vi "GDSProject_CreateFolder.vi"(0 "Project Refnum In":refnum<vi>, 1 "Project Item To Create Folder Below(Use MyComputer if not wired)":refnum<vi>, 3 "FolderName":string, 5 "error in (no error)":errorcluster, 7 "FolderScope":T1(array[ring]), 8 "CreateThePhysicalFolderIfPossible(False)":bool, 9 "GuessFolderScope(False)":bool) -> (14 "Project Refnum Out":refnum<vi>, 15 "ItemOut":refnum<vi>, 16 "FolderCreated":bool, 19 "error out":errorcluster)   [LabVIEW 2020]
panel:
  # "E.g. Private/SubPrivate"
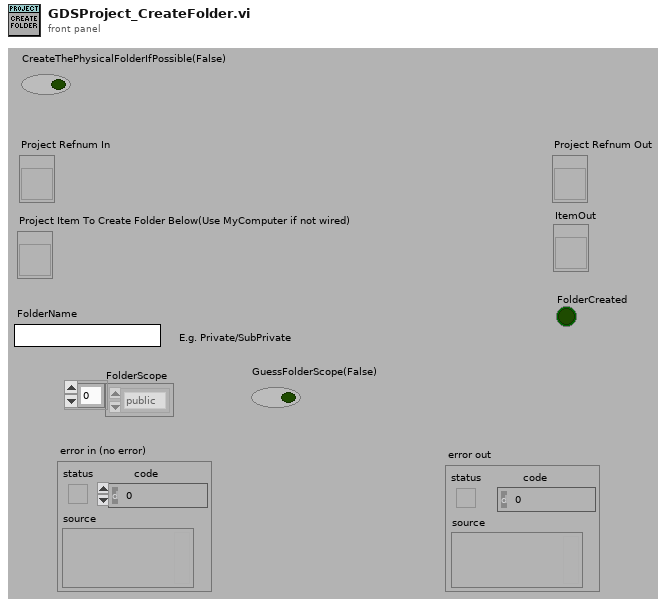
[diagram p1: front panel]
types:
  T1 = enum32{"invalid scope", "public", "private", "protected", "community"}[]
  T2 = enum32{"invalid scope", "public", "private", "protected"}
  T3 = enum32{"invalid scope", "public", "private", "protected", "community"}
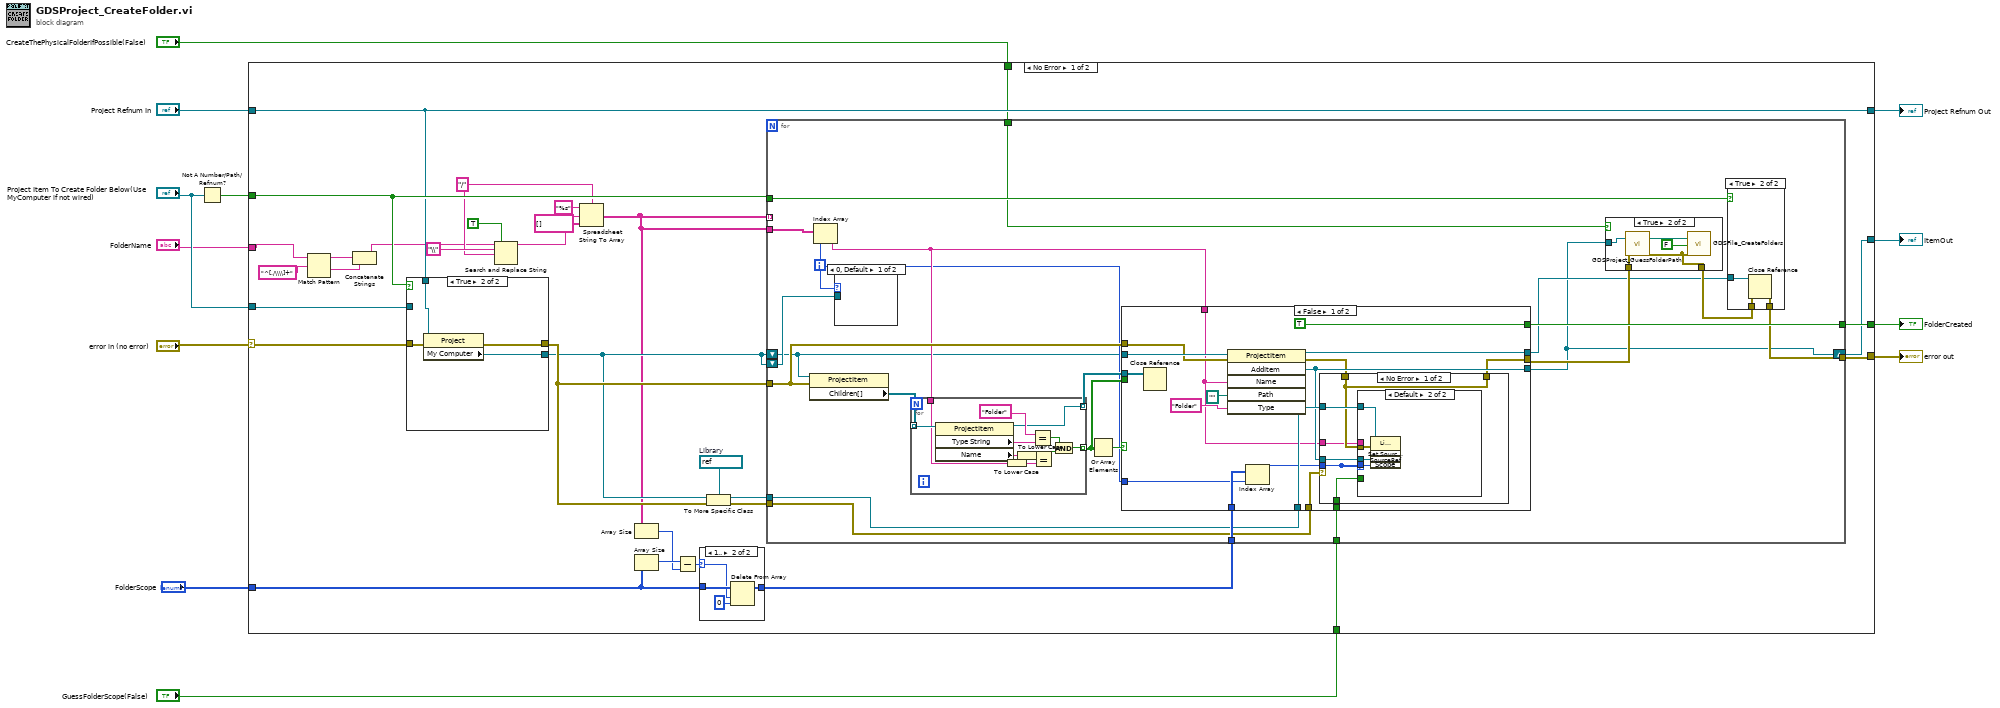
[diagram p0: block diagram]
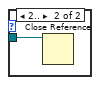
[diagram p3: hidden frame]
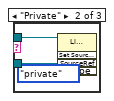
[diagram p7: hidden frame]
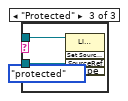
[diagram p8: hidden frame]
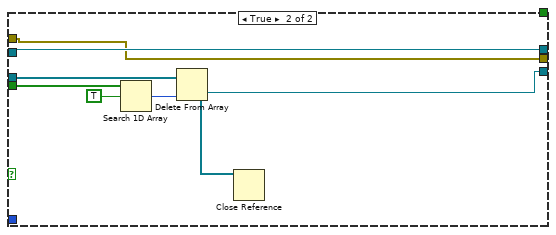
[diagram p10: hidden frame]
diagram:
  n1 = Not A Number/Path/Refnum?(number/path/refnum="Project Item To Create Folder Below(Use MyComputer if not wired)") -> (NaN/Path/Refnum?=w9:bool)
  n2 = case shown="No Error" "error in (no error)" {
    selector: "error in (no error)" -> [w43 w149]
    tunnel: [w37 w149] -> w11
    tunnel: "Project Refnum In" -> [w40 w148]
    tunnel: w9 -> [w41 _]
    tunnel: "Project Item To Create Folder Below(Use MyComputer if not wired)" -> [w42 _]
    tunnel: [w40 w148] -> w7
    tunnel: "FolderName" -> [w20 _]
    tunnel: [w34 _] -> w5
    tunnel: [w39 _] -> w4
    tunnel: "CreateThePhysicalFolderIfPossible(False)" -> [w38 _]
    tunnel: "FolderScope" -> [w13 _]
    tunnel: "GuessFolderScope(False)" -> [w24 _]
    frame No Error {
      w29 = refnum<vi> refnum  # Library
      w32 = "/" ("delimiter (Tab)")
      n3 = Match Pattern(string=w20, regular expression="^[./\\\\]+") -> (before substring=w22:string, after substring=w21:string)  [unwired: 1 in, 2 out]
      n4 = Concatenate Strings(w22, w21) -> (w19:string)
      n5 = case shown="True" w41 {
        tunnel: w40 -> [_ w147]
        tunnel: w43 -> [w142 w146]
        tunnel: [w143 w145] -> w25
        tunnel: w42 -> [w143 _]
        tunnel: [w142 w144] -> w26
        frame False {
        }
        frame True {
          n6 = property class="Project"(reference=w147, error in=w146) -> (error out=w144:errorcluster, "My Computer"=w145:refnum<vi>)  [unwired: 1 out]
        }
      }
      n7 = Search and Replace String(replace all?=TRUE ("replace all? (F)"), input string=w19, search string="\\", replace string=w32) -> (result string=w30:string)  [unwired: 4 in, 3 out]
      n8 = Spreadsheet String To Array(delimiter (Tab)=w32, format string="%s", spreadsheet string=w30, array type (2D Dbl)=string[] []) -> (array=w18:string[])
      n9 = Array Size(array=w18) -> (size(s)=w16:i32)
      n10 = Array Size(array=w13) -> (size(s)=w17:i32)
      n11 = Subtract(x=w17, y=w16) -> (x-y=w14:i32)
      n12 = case shown="1.." w14 {
        selector: w14 -> [_ w45]
        tunnel: w13 -> [w44 w48]
        tunnel: [w44 w47] -> w15
        frame 0, Default {
        }
        frame 1.. {
          n13 = Delete From Array(array=w48, length=w45, index=0) -> (array with subset deleted=w47:T1)  [unwired: 1 out]
        }
      }
      n14 = To More Specific Class(target class=w29, reference=w25, error in=w26) -> (specific class reference=w28:refnum<vi>, error out=w27:errorcluster)
      n15 = for {
        tunnel: w41 -> [w70]
        tunnel: w26 -> [w69]
        tunnel: [w64] -> w39
        tunnel: w38 -> [w63]
        tunnel: [w60] -> w37
        tunnel: w18 -> [_] mode=indexing
        tunnel: w18 -> [w58]
        shift-right: [w56] -> w34
        shift-left: w25 -> [w52]
        shift-left: w25 -> [w55]
        tunnel: w15 -> [w54]
        tunnel: w28 -> [w51]
        tunnel: w27 -> [w50]
        tunnel: w24 -> [w49]
        i -> [w53]
        n16 = property class="ProjectItem"(reference=w52, error in=w69) -> ("Children[]"=w68:refnum<vi>[])  [unwired: 2 out]
        n17 = Index Array(array=w58, index=w53) -> (element=w57:string)
        n18 = case shown="0, Default" w53 {
          tunnel: w55 -> [_ w71]
          frame 0, Default {
          }
          frame 2.. {
            n19 = Close Reference(reference=w71) -> ()  [unwired: 1 in, 1 out]
          }
        }
        n20 = for {
          tunnel: w68 -> [w137] mode=indexing
          tunnel: w57 -> [w133]
          tunnel: [w130] -> w66 mode=indexing
          tunnel: [w129] -> w65 mode=indexing
          n21 = property class="ProjectItem"(reference=w137) -> (reference out=w129:refnum<vi>, "Type String"=w136:string, "Name"=w134:string)  [unwired: 1 in, 1 out]
          n22 = To Lower Case(string=w133) -> (all lower case string=w127:string)
          n23 = To Lower Case(string=w134) -> (all lower case string=w128:string)
          n24 = Equal?(x="Folder", y=w136) -> (x = y?=w132:bool)
          n25 = Equal?(x=w128, y=w127) -> (x = y?=w131:bool)
          n26 = And(x=w132, y=w131) -> (x .and. y?=w130:bool)
        }
        n27 = Or Array Elements(Boolean array=w66) -> (logical OR=w67:bool)
        n28 = case shown="False" w67 {
          tunnel: [w81 w120] -> w62
          tunnel: [w84 w122] -> w56
          tunnel: [w93 w121] -> w59
          tunnel: w52 -> [w91 w121]
          tunnel: w69 -> [w90 w120]
          tunnel: w57 -> [w79 _]
          tunnel: w66 -> [_ w126]
          tunnel: w65 -> [w78 w124]
          tunnel: [TRUE _] -> w64
          tunnel: w54 -> [w88 _]
          tunnel: w53 -> [w87 _]
          tunnel: w50 -> [w86 _]
          tunnel: w51 -> [w85 _]
          tunnel: w49 -> [w80 _]
          frame False {
            n29 = Close Reference(reference=w78) -> ()  [unwired: 1 in, 1 out]
            n30 = invoke class="ProjectItem" method="AddItem"(reference=w91, error in=w90, "Name"=w79, "Path"=path "", "Type"="Folder") -> (reference out=w93:refnum<vi>, error out=w82:errorcluster, "AddItem"=w84:refnum<vi>)  [unwired: 1 in, 3 out]
            n31 = Index Array(array=w88, index=w87) -> (element=w83:T3)
            n32 = case shown="No Error" w86 {
              tunnel: w85 -> [w100 _]
              tunnel: w84 -> [w99 _]
              tunnel: w83 -> [w98 _]
              tunnel: w82 -> [w97 w118]
              tunnel: [w97 w118] -> w81
              tunnel: w80 -> [w96 _]
              tunnel: w79 -> [w95 _]
              frame No Error {
                n33 = case shown="Default" w98 {
                  tunnel: w100 -> [w102 w117]
                  tunnel: w99 -> [w103 w116]
                  tunnel: w97 -> [_ w115]
                  tunnel: w98 -> [_ w114]
                  tunnel: w96 -> [w104 _]
                  tunnel: w95 -> [w101 _]
                  frame "invalid scope" {
                    n34 = case shown="False" w104 {
                      tunnel: w103 -> [_ w106]
                      tunnel: w102 -> [_ w107]
                      tunnel: w101 -> [_ w105]
                      frame False {
                      }
                      frame True {
                        n35 = case shown="\"False\", Default" w105 {
                          tunnel: w107 -> [_ w110 w113]
                          tunnel: w106 -> [_ w109 w112]
                          frame "False", Default {
                          }
                          frame "Private" {
                            n36 = invoke class="Library" method="Set Source Scope"(reference=w110, "SourceRef"=w109, "Scope"=T2."private" ("scope")) -> ()  [unwired: 2 in, 5 out]
                          }
                          frame "Protected" {
                            n37 = invoke class="Library" method="Set Source Scope"(reference=w113, "SourceRef"=w112, "Scope"=T2."protected" ("scope")) -> ()  [unwired: 2 in, 5 out]
                          }
                        }
                      }
                    }
                  }
                  frame Default {
                    n38 = invoke class="Library" method="Set Source Scope"(reference=w117, error in=w115, "SourceRef"=w116, "Scope"=w114) -> ()  [unwired: 1 in, 5 out]
                  }
                }
              }
              frame Error {
              }
            }
          }
          frame True {
            n39 = Search 1D Array(1D array=w126, element=TRUE) -> (index of element=w123:i32)  [unwired: 1 in]
            n40 = Delete From Array(array=w124, index=w123) -> (deleted portion=w122:refnum<vi>, array with subset deleted=w119:refnum<vi>[])  [unwired: 1 in]
            n41 = Close Reference(reference=w119) -> ()  [unwired: 1 in, 1 out]
          }
        }
        n42 = case shown="True" w63 {
          tunnel: w62 -> [w72 w76]
          tunnel: [w72 w75] -> w61
          tunnel: w56 -> [_ w73]
          frame False {
          }
          frame True {
            n43 = call "GDSProject_GuessFolderPath.vi"("ProjectItem"=w73, "error in (no error)"=w76) -> ("Path"=w77:path, "error out"=w75:errorcluster)  [unwired: 14 in, 2 out]
            n44 = call "GDSFile_CreateFolders.vi"("Path"=w77, "Promt if folder\ndoes not exists?"=FALSE ("Promt if folder\ndoes not exists?"), "error in (no error)"=w75) -> ()  [unwired: 12 in, 5 out]
          }
        }
        n45 = case shown="True" w70 {
          tunnel: [w138 w141] -> w60
          tunnel: w59 -> [_ w140]
          tunnel: w61 -> [w138 w139]
          frame False {
          }
          frame True {
            n46 = Close Reference(reference=w140, error in (no error)=w139) -> (error out=w141:errorcluster)
          }
        }
      }
    }
    frame Error {
    }
  }
  "Project Refnum Out" <- w7
  "error out" <- w11
  "ItemOut" <- w5
  "FolderCreated" <- w4
